vi "C_Decode_To_Frames.vi"(8 "error in (no error)":errorcluster, 9 "bytes in":u8[](array[numeric]), 10 "frames in":T2 {"flags" format="%.0x"; "id" format="%.0x"}, 11 "state in":T1) -> (0 "error out":errorcluster, 1 "result":T3, 2 "frames out":T2 {"flags" format="%.0x"; "id" format="%.0x"}, 3 "state out":T1)   [LabVIEW 2021, in "CANsub_API.lvlib"]
doc: "API private: decodes WebSocket bytes into the caller’s CANsub_Frames in place (csb_decode_ws_to_can); decoder state (ws, hdlc, ping) kept in C_RX_State; sets frames.count = n frames. Capacity = size of frames.id. With an error in: count 0, nothing decoded."
uses:
  CANsub_API.lvlib
  C_Decode_Result.ctl
  CANsub_C.lvlib
  codec_vis/CANsub_Codec.lvlib
  C_RX_State.ctl
  Typedefs/CANsub_Frames.ctl
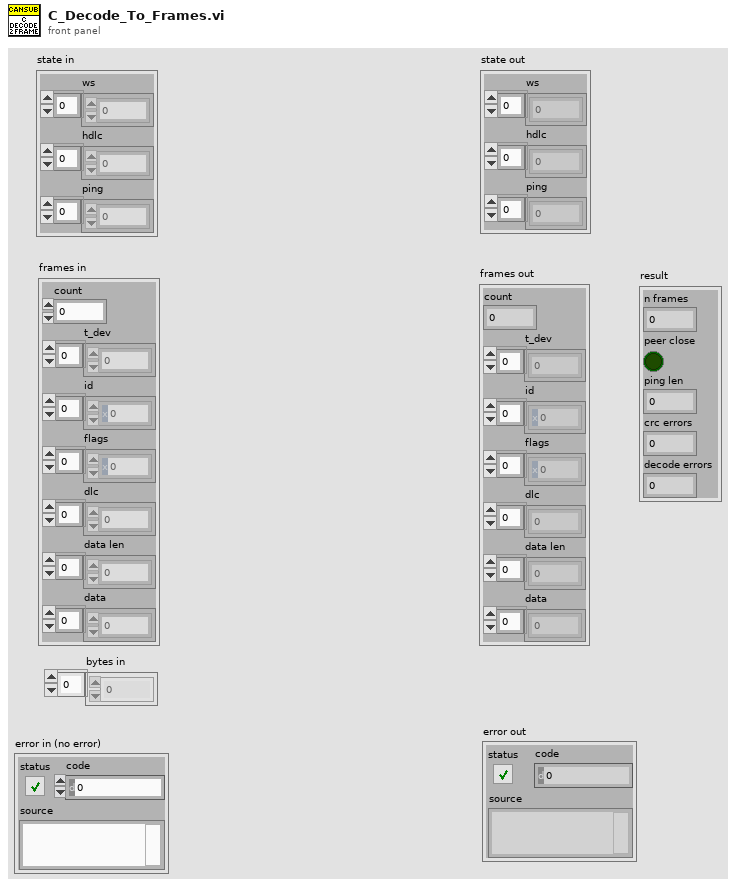
[diagram p1: front panel]
types:
  T1 = typedef "CANsub_C.lvlib/C_RX_State.ctl" = cluster{"ws":u8[], "hdlc":u8[], "ping":u8[]}
  T2 = typedef "CANsub_API.lvlib/CANsub_Frames.ctl" = cluster{"count":i32, "t_dev":dbl[], "id":u32[], "flags":u16[], "dlc":u8[], "data len":u8[], "data":u8[]}
  T3 = typedef "CANsub_C.lvlib/C_Decode_Result.ctl" = cluster{"n frames":i32, "peer close":bool, "ping len":i32, "crc errors":u32, "decode errors":i32}
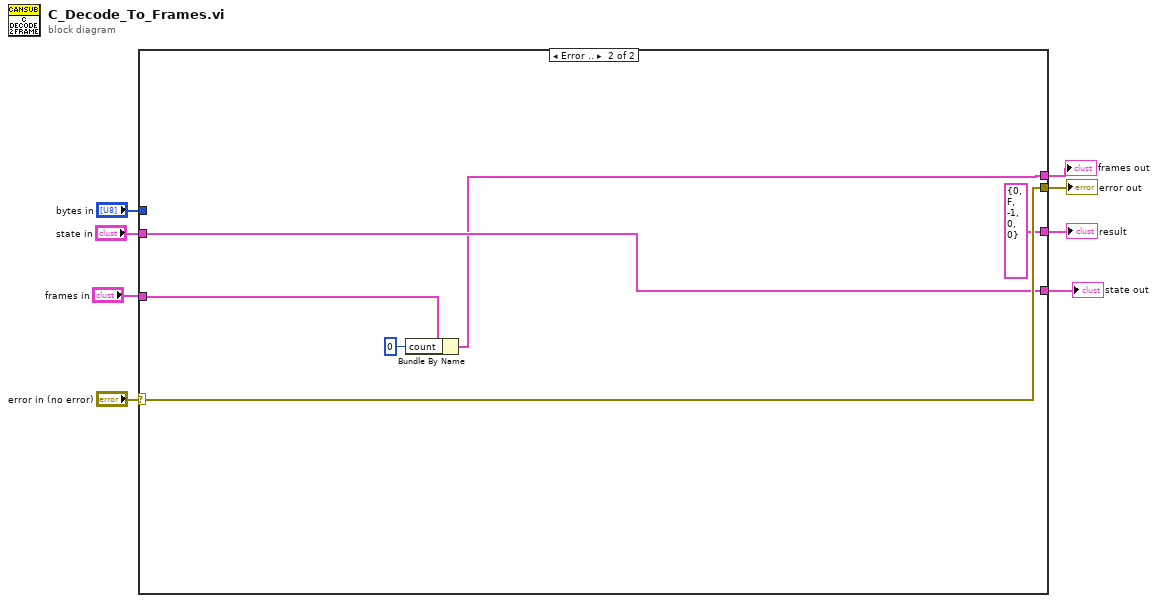
[diagram p0: block diagram]
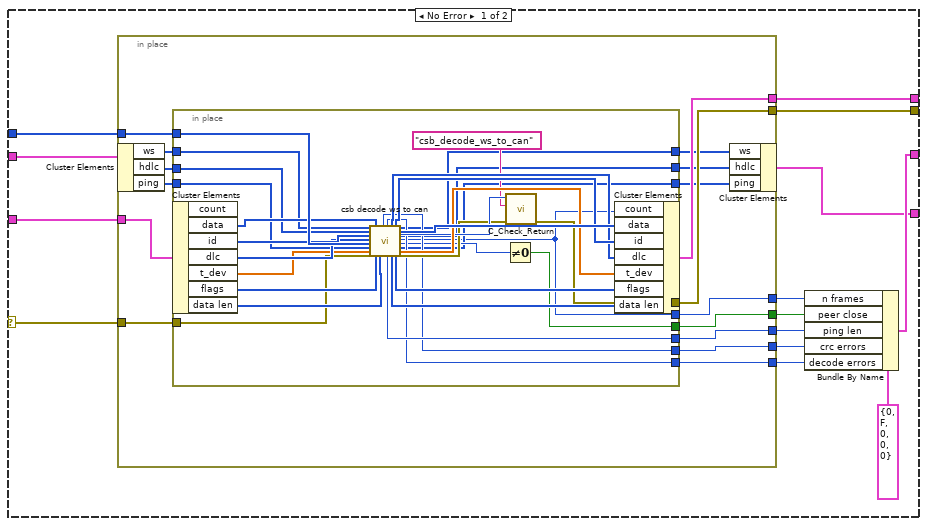
[diagram p2: hidden frame]
diagram:
  n1 = case shown="Error .." "error in (no error)" {
    selector: "error in (no error)" -> [w20 w74]
    tunnel: [w11 w74] -> w7
    tunnel: [w19 w69] -> w2
    tunnel: "frames in" -> [w22 w71]
    tunnel: [w12 T3 {"n frames"=0, "peer close"=FALSE, "ping len"=-1, "crc errors"=0, "decode errors"=0} ("result")] -> w6
    tunnel: "bytes in" -> [w21 _]
    tunnel: "state in" -> [w10 w72]
    tunnel: [w9 w72] -> w1
    frame No Error {
      n2 = in-place {
        in-place-border: w22 -> [w38]
        in-place-border: w21 -> [w37]
        in-place-border: w20 -> [w36]
        in-place-border: [w35] -> w19
        in-place-border: [w34] -> w17
        in-place-border: [w33] -> w16
        in-place-border: [w32] -> w15
        in-place-border: [w31] -> w14
        in-place-border: [w30] -> w13
        in-place-border: [w29] -> w11
        n3 = in-place-cluster #1(w10) -> ("ws"=w28:u8[], "hdlc"=w27:u8[], "ping"=w26:u8[])
        n4 = in-place {
          in-place-border: w37 -> [w68]
          in-place-border: w36 -> [w62]
          in-place-border: [w51] -> w34
          in-place-border: [w50] -> w33
          in-place-border: [w49] -> w32
          in-place-border: [w39] -> w31
          in-place-border: [w47] -> w30
          in-place-border: [w46] -> w29
          in-place-border: w28 -> [w45]
          in-place-border: w27 -> [w44]
          in-place-border: w26 -> [w43]
          in-place-border: [w42] -> w25
          in-place-border: [w41] -> w24
          in-place-border: [w40] -> w23
          n5 = in-place-cluster #2(w38) -> ("data"=w61:u8[], "id"=w67:u32[], "dlc"=w66:u8[], "t_dev"=w65:dbl[], "flags"=w64:u16[], "data len"=w63:u8[])  [unwired: 1 out]
          n6 = call "csb decode ws to can.vi"("ws_state"=w45, "hdlc_state"=w44, "id"=w67, "dlc"=w66, "in"=w68, "ping_payload"=w43, "t_dev"=w65, "error in (no error)"=w62, "data"=w61, "flags"=w64, "data_len"=w63) -> ("function return"=w54:i32, "crc_errors"=w50:u32, "decode_errors"=w49:i32, "ping_len"=w51:i32, "dlc out"=w55:u8[], "data_len out"=w57:u8[], "id out"=w56:u32[], "flags out"=w58:u16[], "ws_state out"=w42:u8[], "data out"=w60:u8[], "hdlc_state out"=w41:u8[], "n_frames"=w39:i32, "peer_close"=w48:i32, "ping_payload out"=w40:u8[], "t_dev out"=w59:dbl[], "error out"=w53:errorcluster)  [unwired: 1 in]
          n7 = Not Equal To 0?(x=w48) -> (x != 0?=w47:bool)
          n8 = call "C_Check_Return.vi"("error in (no error)"=w53, "function name"="csb_decode_ws_to_can", "function return"=w54) -> ("error out"=w46:errorcluster)  [unwired: 6 in, 2 out]
          n9 = in-place-cluster #2("count"=w39, "data"=w60, "id"=w56, "dlc"=w55, "t_dev"=w59, "flags"=w58, "data len"=w57) -> (w35:T2)
        }
        n10 = in-place-cluster #1("ws"=w25, "hdlc"=w24, "ping"=w23) -> (w9:T1)
      }
      n11 = Bundle By Name(cluster=T3 {"n frames"=0, "peer close"=FALSE, "ping len"=0, "crc errors"=0, "decode errors"=0} ("C_Decode_Result"), "n frames"=w14, "peer close"=w13, "ping len"=w17, "crc errors"=w16, "decode errors"=w15) -> (w12:T3)
    }
    frame Error {
      n12 = Bundle By Name(cluster=w71, "count"=0) -> (w69:T2)
    }
  }
  "result" <- w6
  "error out" <- w7
  "frames out" <- w2
  "state out" <- w1
